vi "ton.vi"(10 "Time":i32, 11 "START":bool) -> (2 "ET":i32, 3 "Q":bool)   [LabVIEW 2020]
panel:
  out "Time 2":i32
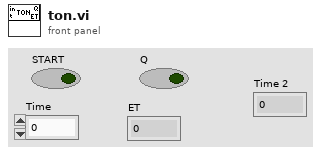
[diagram p1: front panel]
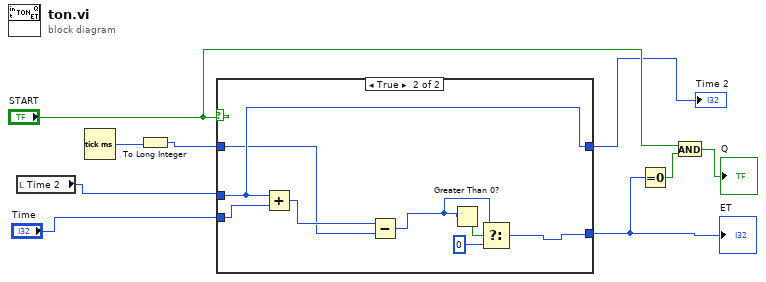
[diagram p0: block diagram]
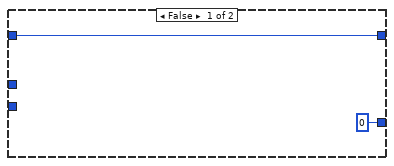
[diagram p2: hidden frame]
diagram:
  n1 = local read "Time 2"() -> (w1:i32)
  n2 = Tick Count (ms)() -> (millisecond timer value=w5:u32)
  n3 = To Long Integer(number=w5) -> (32bit integer=w4:i32)
  n4 = case shown="True" "START" {
    tunnel: w4 -> [w11 w16]
    tunnel: [w11 w19] -> w2
    tunnel: w1 -> [_ w19]
    tunnel: "Time" -> [_ w18]
    tunnel: [0 ("f") w13] -> w3
    frame False {
    }
    frame True {
      n5 = Add(x=w19, y=w18) -> (x+y=w17:i32)
      n6 = Subtract(x=w17, y=w16) -> (x-y=w14:i32)
      n7 = Greater Than 0?(x=w14) -> (x > 0?=w15:bool)
      n8 = Select(t=w14, s=w15, f=0) -> (s? t:f=w13:i32)
    }
  }
  "ET" <- w3
  "Time 2" <- w2
  n9 = Equal To 0?(x=w3) -> (x = 0?=w7:bool)
  n10 = And(x="START", y=w7) -> (x .and. y?=→"Q":bool)
